vi "test Decode Parameters for Labels in a Channel.vi"(8 "error in":errorcluster, 11 "TestCase in":refnum<class "Engine.lvclass">) -> (0 "error out":errorcluster, 3 "TestCase out":refnum<class "Engine.lvclass">)   [LabVIEW 2020, in "Engine.lvclass"]
uses:
  Engine.lvclass
  Shared/RT Label Settings.ctl
  Shared/Label.ctl
  Shared/RT Parameters.ctl
  Shared/Parameter Definition.ctl
  <vilib>/NI/NI VeriStand Encoding and Decoding/Encoding.ctl
  <vilib>/NI VeriStand/Custom Device API/Custom Device Item Ref.ctl
  Shared/Transfer Type.ctl
  <vilib>/NI VeriStand/Custom Device API/Data Reference.ctl
  <vilib>/addons/_JKI Toolkits/VI Tester/TestCase.llb/TestCase.lvclass
  Engine/Implementation/Rx Execution Unit/Rx Execution Unit.lvclass
  <vilib>/NI VeriStand/Custom Device API/Custom Device API.lvlib
  <vilib>/NI/NI VeriStand Encoding and Decoding/Encoding and Decoding.lvlib
  C:/Program Files (x86)/National Instruments/LabVIEW 2020/vi.lib/addons/_JKI Toolkits/VI Tester/TestCase.llb/TestCase.lvclass
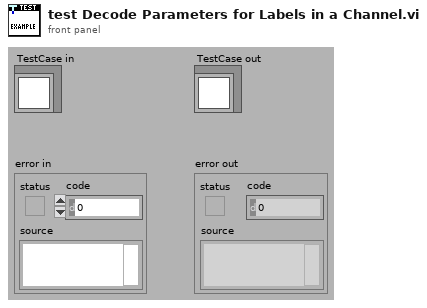
[diagram p1: front panel]
types:
  T1 = typedef "RT Label Settings.ctl" = cluster{"Name":string, "xmlName":string, "label":T2, "transfer period":u32, "SDI_Enabled":bool, "SDI":u8, "parameter driver data":T3, "transfer type":T7, "has timestamp?":bool, "Label Disable/Trigger Channel Reference":T6, "Message Handle":u64, "Initialized?":bool, "Word Initial Raw Value":u32, "Label Timestamp Channel Data Reference":T8, "disabled":bool, "modified":bool}
  T2 = typedef "Label.ctl" = u8
  T3 = typedef "RT Parameters.ctl" = cluster{"parameter definitions":T4[], "Tx parameter refs":T6[]}
  T4 = typedef "Parameter Definition.ctl" = cluster{"start index":i32, "size":i32, "encoding":T5, "signed":bool, "scale multiplier":dbl, "scale offset":dbl, "default value":dbl}
  T5 = typedef "Encoding and Decoding.lvlib/Encoding.ctl" = enum16{"BNR", "BCD", "Discrete"}
  T6 = typedef "Custom Device API.lvlib/Custom Device Item Ref.ctl" = u64
  T7 = typedef "Transfer Type.ctl" = enum16{"Scheduled", "Acyclic", "Block", "Strobe"}
  T8 = typedef "Custom Device API.lvlib/Data Reference.ctl" = i32
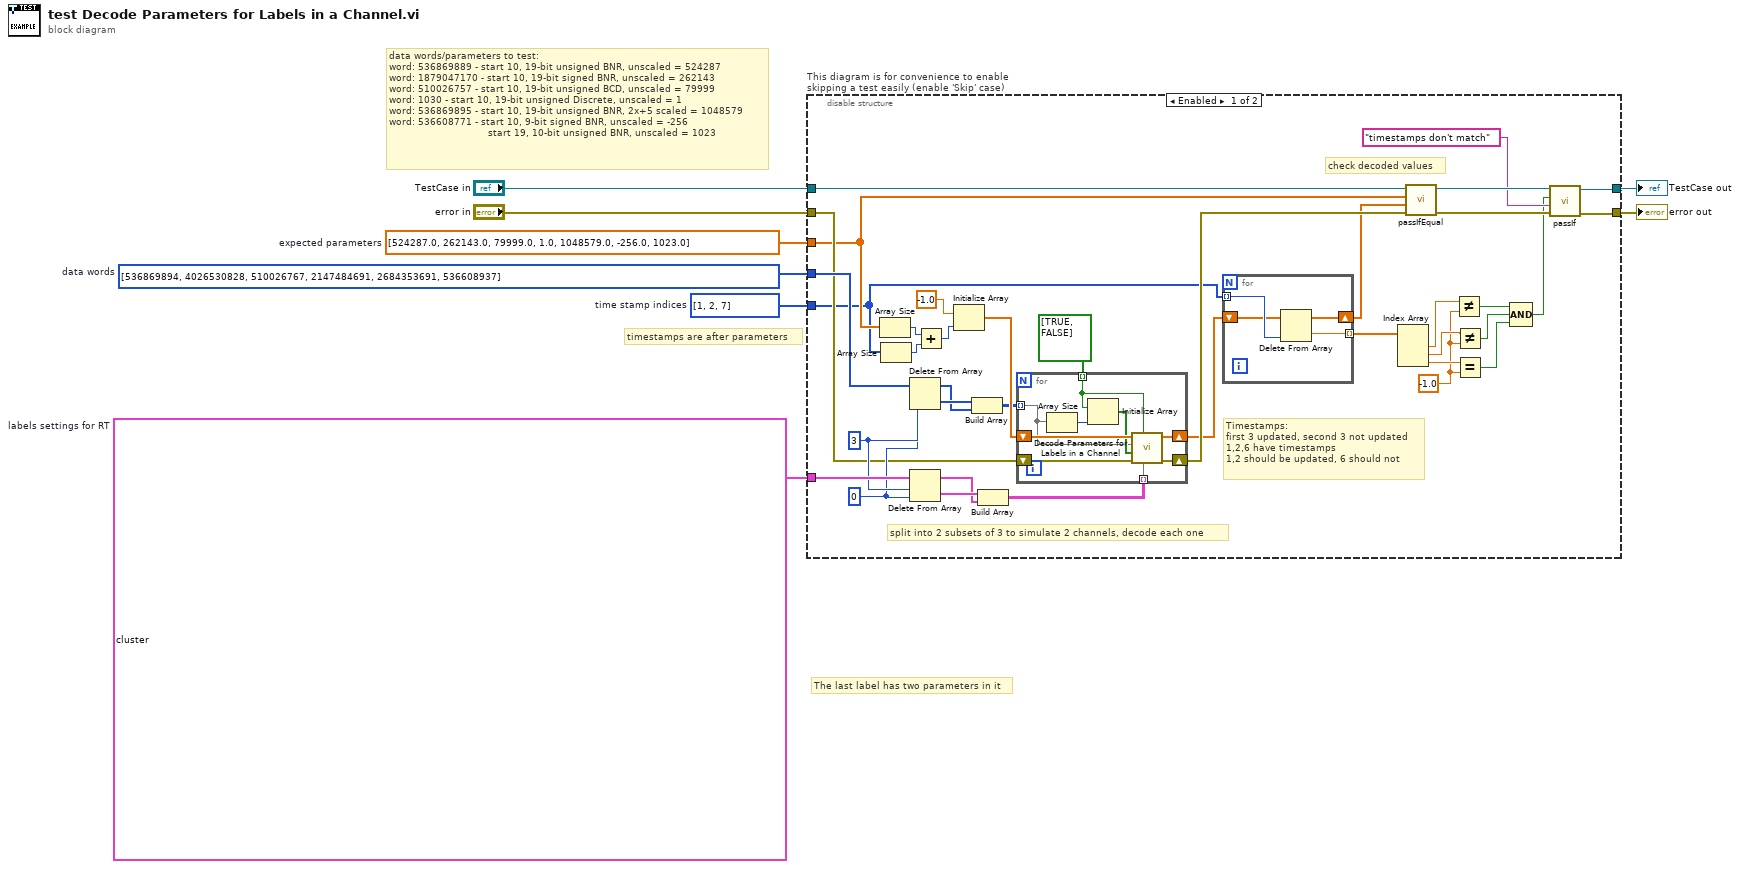
[diagram p0: block diagram]
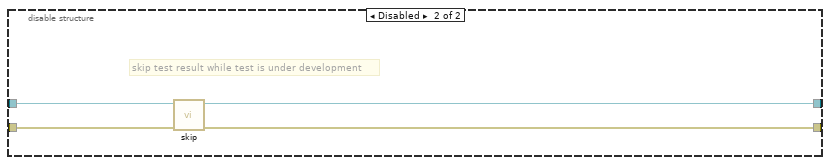
[diagram p2: hidden frame]
diagram:
  w1 = i32[] [1, 2, 7]  # time stamp indices
  w3 = dbl[] [524287.0, 262143.0, 79999.0, 1.0, 1048579.0, -256.0, 1023.0]  # expected parameters
  w4 = T1[] [{"Name"="", "xmlName"="", "label"=0, "transfer period"=0, "SDI_Enabled"=FALSE, "SDI"=0, "parameter driver data"={"parameter definitions"=[{"start index"=10, "size"=19, "encoding"=enum."BNR", "signed"=FALSE, "scale multiplier"=1.0, "scale offset"=0.0, "default value"=0.0}], "Tx parameter refs"=[]}, "transfer type"=enum."Scheduled", "has timestamp?"=TRUE, "Label Disable/Trigger Channel Reference"=0, "Message Handle"=0, "Initialized?"=FALSE, "Word Initial Raw Value"=0, "Label Timestamp Channel Data Reference"=0, "disabled"=FALSE, "modified"=FALSE}, {"Name"="", "xmlName"="", "label"=0, "transfer period"=0, "SDI_Enabled"=FALSE, "SDI"=0, "parameter driver data"={"parameter definitions"=[{"start index"=10, "size"=19, "encoding"=enum."BNR", "signed"=TRUE, "scale multiplier"=1.0, "scale offset"=0.0, "default value"=0.0}], "Tx parameter refs"=[]}, "transfer type"=enum."Scheduled", "has timestamp?"=TRUE, "Label Disable/Trigger Channel Reference"=0, "Message Handle"=0, "Initialized?"=FALSE, "Word Initial Raw Value"=0, "Label Timestamp Channel Data Reference"=0, "disabled"=FALSE, "modified"=FALSE}, {"Name"="", "xmlName"="", "label"=0, "transfer period"=0, "SDI_Enabled"=FALSE, "SDI"=0, "parameter driver data"={"parameter definitions"=[{"start index"=10, "size"=19, "encoding"=enum."BCD", "signed"=FALSE, "scale multiplier"=1.0, "scale offset"=0.0, "default value"=0.0}], "Tx parameter refs"=[]}, "transfer type"=enum."Scheduled", "has timestamp?"=FALSE, "Label Disable/Trigger Channel Reference"=0, "Message Handle"=0, "Initialized?"=FALSE, "Word Initial Raw Value"=0, "Label Timestamp Channel Data Reference"=0, "disabled"=FALSE, "modified"=FALSE}, {"Name"="", "xmlName"="", "label"=0, "transfer period"=0, "SDI_Enabled"=FALSE, "SDI"=0, "parameter driver data"={"parameter definitions"=[{"start index"=10, "size"=19, "encoding"=enum."Discrete", "signed"=FALSE, "scale multiplier"=1.0, "scale offset"=0.0, "default value"=0.0}], "Tx parameter refs"=[]}, "transfer type"=enum."Scheduled", "has timestamp?"=FALSE, "Label Disable/Trigger Channel Reference"=0, "Message Handle"=0, "Initialized?"=FALSE, "Word Initial Raw Value"=0, "Label Timestamp Channel Data Reference"=0, "disabled"=FALSE, "modified"=FALSE}, {"Name"="", "xmlName"="", "label"=0, "transfer period"=0, "SDI_Enabled"=FALSE, "SDI"=0, "parameter driver data"={"parameter definitions"=[{"start index"=10, "size"=19, "encoding"=enum."BNR", "signed"=FALSE, "scale multiplier"=2.0, "scale offset"=5.0, "default value"=0.0}], "Tx parameter refs"=[]}, "transfer type"=enum."Scheduled", "has timestamp?"=FALSE, "Label Disable/Trigger Channel Reference"=0, "Message Handle"=0, "Initialized?"=FALSE, "Word Initial Raw Value"=0, "Label Timestamp Channel Data Reference"=0, "disabled"=FALSE, "modified"=FALSE}, {"Name"="", "xmlName"="", "label"=0, "transfer period"=0, "SDI_Enabled"=FALSE, "SDI"=0, "parameter driver data"={"parameter definitions"=[{"start index"=10, "size"=9, "encoding"=enum."BNR", "signed"=TRUE, "scale multiplier"=1.0, "scale offset"=0.0, "default value"=0.0}, {"start index"=19, "size"=10, "encoding"=enum."BNR", "signed"=FALSE, "scale multiplier"=1.0, "scale offset"=0.0, "default value"=0.0}], "Tx parameter refs"=[]}, "transfer type"=enum."Scheduled", "has timestamp?"=TRUE, "Label Disable/Trigger Channel Reference"=0, "Message Handle"=0, "Initialized?"=FALSE, "Word Initial Raw Value"=0, "Label Timestamp Channel Data Reference"=0, "disabled"=FALSE, "modified"=FALSE}]  # labels settings for RT
  w5 = u32[] [536869894, 4026530828, 510026767, 2147484691, 2684353691, 536608937]  # data words
  # "timestamps are after parameters"
  # "The last label has two parameters in it"
  # "for visibility, irrelevant label settings are minimized in this constant"
  # "data words/parameters to test:\nword: 536869889 - start 10, 19-bit unsigned BNR, unscaled = 524287\nword: 1879047170 - start 10, 19-bit signed BNR, unscaled = 262143\nword: 510026757 - start 10, 19-bit unsigned BCD, unscaled = 79999\nword: 1030 - start 10, 19-bit unsigned Discrete, unscaled = 1\nword: 536869895 - start 10, 19-bit unsigned BNR, 2x+5 scaled = 1048579 \nword: 536608771 - start 10, 9-bit signed BNR, unscaled = -256\n                                 start 19, 10-bit unsigned BNR, unscaled = 1023"
  n1 = disable-structure "This diagram is for convenience to enable skipping a test easily (enable 'Skip' case)" shown="Enabled" {
    disable-tunnel: "TestCase in" -> [w43 w62]
    disable-tunnel: [w30 w60] -> w2
    disable-tunnel: [w32 w61] -> w7
    disable-tunnel: "error in" -> [w40 w59]
    disable-tunnel: w5 -> [w44 _]
    disable-tunnel: w4 -> [w45 _]
    disable-tunnel: w3 -> [w36 _]
    disable-tunnel: w1 -> [w27 _]
    frame Enabled {
      w20 = -1.0
      w41 = 0 ("index")
      w42 = 3 ("length")
      # "Timestamps: \nfirst 3 updated, second 3 not updated\n1,2,6 have timestamps\n1,2 should be updated, 6 should not"
      # "check decoded values"
      # "split into 2 subsets of 3 to simulate 2 channels, decode each one"
      n2 = Array Size(array=w36) -> (size(s)=w25:i32)
      n3 = Array Size(array=w27) -> (size(s)=w26:i32)
      n4 = Delete From Array(array=w44, length=w42, index=w41) -> (deleted portion=w14:u32[], array with subset deleted=w13:u32[])
      n5 = Delete From Array(array=w45, length=w42, index=w41) -> (deleted portion=w11:T1[], array with subset deleted=w10:T1[])
      n6 = Add(x=w25, y=w26) -> (x+y=w24:i32)
      n7 = Initialize Array(-1.0 ("element"), w24) -> (w37:dbl[])
      n8 = Build Array(w14, w13) -> (w12:u32[][])
      n9 = Build Array(w11, w10) -> (w9:T1[][])
      n10 = for {
        tunnel: bool[] [TRUE, FALSE] ("reset index") -> [w48] mode=indexing
        tunnel: w12 -> [w47] mode=indexing
        tunnel: w9 -> [w46] mode=indexing
        shift-right: [w53] -> w39
        shift-left: w40 -> [w54]
        shift-right: [w51] -> w35
        shift-left: w37 -> [w52]
        n11 = Array Size(array=w47) -> (size(s)=w50:i32)
        n12 = Initialize Array(w48, w50) -> (w49:bool[])
        n13 = call "Decode Parameters for Labels in a Channel.vi"("labels settings for RT"=w46, "reset index"=w48, "error in (no error)"=w54, "updated labels?"=w49, "data words in"=w47, "Parameter Values in"=w52) -> ("error out"=w53:errorcluster, "Parameter Values out"=w51:dbl[])  [unwired: 4 in]
      }
      n14 = for {
        tunnel: w27 -> [w58] mode=indexing
        shift-right: [w56] -> w28
        shift-left: w35 -> [w57]
        tunnel: [w55] -> w34 mode=indexing
        n15 = Delete From Array(array=w57, index=w58) -> (deleted portion=w55:dbl, array with subset deleted=w56:dbl[])  [unwired: 1 in]
      }
      n16 = Index Array(array=w34) -> (element #1=w23:dbl, element #2=w22:dbl, element #3=w21:dbl)  [unwired: 3 in]
      n17 = call-dynamic "passIfEqual.vi"("error in (no error)"=w39, "y"=w28, "x"=w36, "TestCase in"=w43) -> ("error out"=w33:errorcluster, "TestCase out"=w31:refnum<class "Engine.lvclass">)  [unwired: 6 in]
      n18 = Not Equal?(x=w23, y=w20) -> (x != y?=w19:bool)
      n19 = Not Equal?(x=w22, y=w20) -> (x != y?=w18:bool)
      n20 = Equal?(x=w21, y=w20) -> (x = y?=w17:bool)
      n21 = Compound Arithmetic op=AND(w19, w18, w17) -> (w16:bool)
      n22 = call-dynamic "passIf.vi"("error in (no error)"=w33, "message (\"\")"="timestamps don't match" ("message (\"\")"), "pass"=w16, "TestCase in"=w31) -> ("error out"=w32:errorcluster, "TestCase out"=w30:refnum<class "Engine.lvclass">)  [unwired: 6 in]
    }
    frame Disabled {
      # "skip test result while test is under development"
      n23 = call <vilib>:"skip.vi"("error in (no error)"=w59, "TestCase in"=w62) -> ("error out"=w61:errorcluster, "TestCase out"=w60:refnum<class "Engine.lvclass">)  [unwired: 8 in]
    }
  }
  "error out" <- w7
  "TestCase out" <- w2
